vi "Initialize UI Elements.vi"(8 "error in":errorcluster, 10 "References":refnum<vi>[](array[refnum]), 11 "NumSlots":i32) -> (0 "error out":errorcluster, 1 "Programming Mode Out":T1[](array[typedef]))   [LabVIEW 2020, in "SEECD System Explorer.lvlib"]
doc: "Initialize Slot Programming Modes Controls (8 elements). We use individual elements because we want to be able to control respective \"Enable State\"."
uses:
  SEECD System Explorer.lvlib
  Type Defs/Slot - Configuration.ctl
  Type Defs/Slot Programming Mode.ctl
panel:
  in  "Slot Programming Mode":T1=enum."Scan Engine"
  in  "Slot 2":string
  in  "Slot":T2={"Slot"="", "Module Name"="", "Current Prog Mode"="", "New Prog Mode"=enum."Scan Engine"}
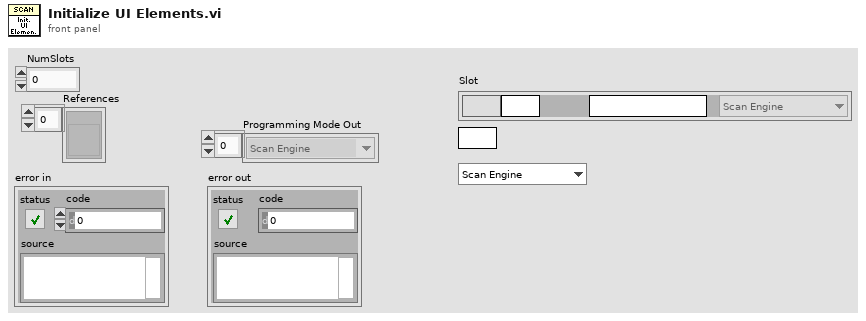
[diagram p1: front panel]
types:
  T1 = typedef "SEECD System Explorer.lvlib/Slot Programming Mode.ctl" = enum16{"Don't Modify", "Scan Engine", "LabVIEW FPGA", "NI-DAQmx"}
  T2 = typedef "SEECD System Explorer.lvlib/Slot - Configuration.ctl" = cluster{"Slot":string, "Module Name":string, "Current Prog Mode":string, "New Prog Mode":T1}
  T3 = enum8{"Enabled", "Disabled", "Disabled and Grayed Out"}
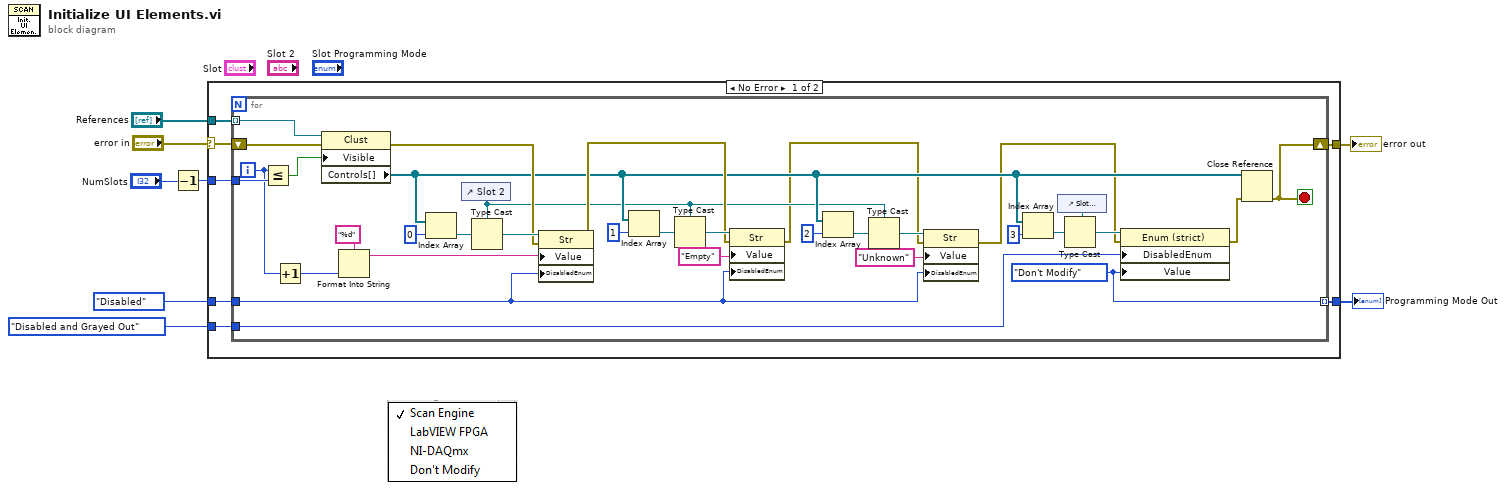
[diagram p0: block diagram]
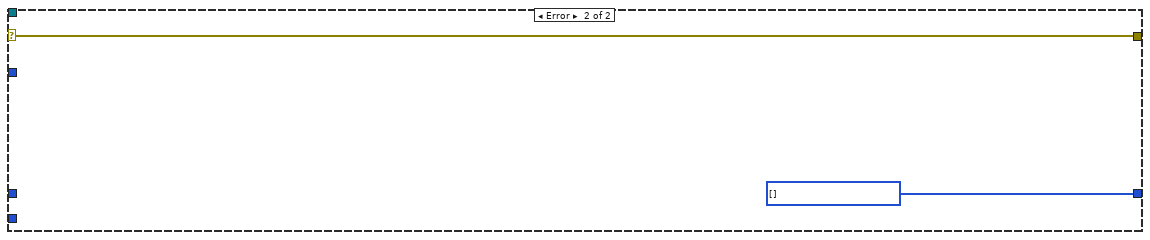
[diagram p2: hidden frame]
diagram:
  n1 = Decrement(x="NumSlots") -> (x-1=w4:i32)
  n2 = case shown="No Error" "error in" {
    selector: "error in" -> [w12 w51]
    tunnel: "References" -> [w15 _]
    tunnel: T3."Disabled" ("Disabled") -> [w14 _]
    tunnel: [w13 w51] -> w7
    tunnel: w4 -> [w11 _]
    tunnel: T3."Disabled and Grayed Out" ("Disabled") -> [w10 _]
    tunnel: [w9 w50] -> w2
    frame No Error {
      n3 = for {
        tunnel: w15 -> [w48] mode=indexing
        shift-right: [w26] -> w13
        shift-left: w12 -> [w47]
        tunnel: w14 -> [w18]
        tunnel: w11 -> [w49]
        tunnel: w10 -> [w31]
        tunnel: [w30] -> w9 mode=indexing
        i -> [w43]
        stop <- w26 stop-if-true
        w30 = Slot_Programming_Mode."Don't Modify" ("Value")
        n4 = Less Or Equal?(x=w43, y=w49) -> (x <= y?=w25:bool)
        n5 = Increment(x=w43) -> (x+1=w42:i32)
        n6 = property class="Clust"(reference=w48, error in=w47, "Visible"=w25) -> (error out=w29:errorcluster, "Controls[]"=w20:refnum<vi>[])  [unwired: 1 out]
        n7 = Format Into String(format string="%d", w42) -> (resulting string=w40:string)  [unwired: 2 in, 1 out]
        n8 = Index Array(array=w20, index=0) -> (element=w45:refnum<vi>)
        n9 = control-ref of="Slot 2"() -> (w19:refnum<vi>)
        n10 = Type Cast(type=w19, x=w45) -> (*(type *) &x=w44:refnum<vi>)
        n11 = property class="Str"(reference=w44, error in=w29, "Value"=w40, "DisabledEnum"=w18) -> (error out=w28:errorcluster)  [unwired: 1 out]
        n12 = Index Array(array=w20, index=1) -> (element=w38:refnum<vi>)
        n13 = Type Cast(type=w19, x=w38) -> (*(type *) &x=w39:refnum<vi>)
        n14 = property class="Str"(reference=w39, error in=w28, "Value"="Empty", "DisabledEnum"=w18) -> (error out=w17:errorcluster)  [unwired: 1 out]
        n15 = Index Array(array=w20, index=2) -> (element=w22:refnum<vi>)
        n16 = Type Cast(type=w19, x=w22) -> (*(type *) &x=w21:refnum<vi>)
        n17 = property class="Str"(reference=w21, error in=w17, "Value"="Unknown", "DisabledEnum"=w18) -> (error out=w16:errorcluster)  [unwired: 1 out]
        n18 = Index Array(array=w20, index=3) -> (element=w33:refnum<vi>)
        n19 = control-ref of="Slot Programming Mode"() -> (w34:refnum<vi>)
        n20 = Type Cast(type=w34, x=w33) -> (*(type *) &x=w32:refnum<vi>)
        n21 = property class="Enum (strict)"(reference=w32, error in=w16, "DisabledEnum"=w31, "Value"=w30) -> (error out=w27:errorcluster)  [unwired: 1 out]
        n22 = Close Reference(reference=w20, error in (no error)=w27) -> (error out=w26:errorcluster)
      }
    }
    frame Error {
      w50 = T1[] [] items=["Don't Modify", "Scan Engine", "LabVIEW FPGA", "NI-DAQmx"]
    }
  }
  "error out" <- w7
  "Programming Mode Out" <- w2
